vi "Demo - plot.vi"() -> ()   [LabVIEW 2021]
uses:
  Apin typedef.ctl
panel:
  in  "Analog pin":T1
  out "Waveform Chart":i32[](graph)
  out "error out":errorcluster
  in  "port":u32
  in  "Base URL":string
  in  "stop":bool
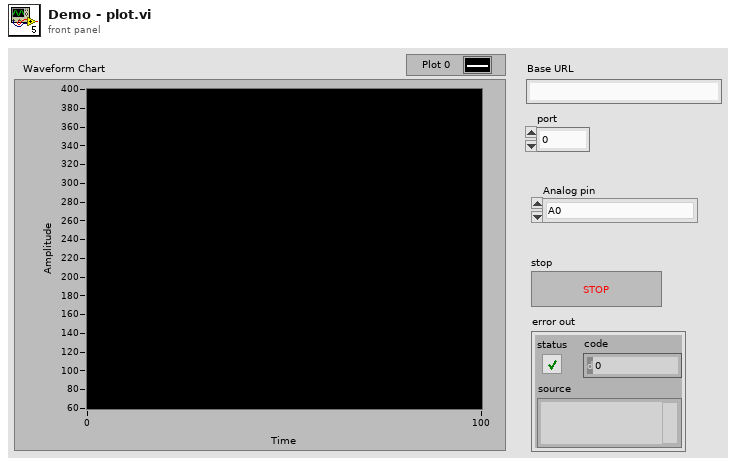
[diagram p1: front panel]
types:
  T1 = typedef "Apin typedef.ctl" = enum16{"A0", "A1", "A2", "A3", "A4", "A5"}
  T2 = typedef "UNO Q Session.ctl" = cluster{"HTTP client":T3, "Base URL":string, "Connected":bool}
  T3 = typedef "LabVIEWHTTPClient.lvlib/ClientHandle.ctl" = refnum<k1>
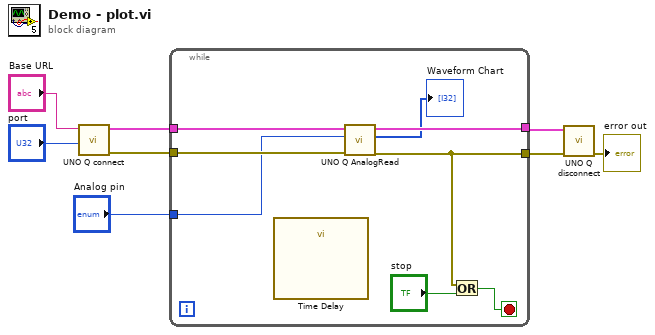
[diagram p0: block diagram]
diagram:
  n1 = call "UNO Q connect.vi"("port"="port", "Base URL"="Base URL") -> ("error out"=w5:errorcluster, "Session out"=w6:T2)  [unwired: 4 in]
  n2 = while {
    tunnel: w6 -> [w15]
    tunnel: w5 -> [w14]
    tunnel: [w16] -> w4
    tunnel: [w9] -> w2
    tunnel: "Analog pin" -> [w12]
    stop <- w11 stop-if-true
    n3 = call "Time Delay"() -> ()  [unwired: 11 in, 1 out]
    n4 = call "UNO Q AnalogRead.vi"("error in (no error)"=w14, "Analog pin"=w12, "UNO Q Session in"=w15) -> ("error out"=w9:errorcluster, "values"=→"Waveform Chart":i32[], "UNO Q Session out"=w16:T2)  [unwired: 4 in, 2 out]
    n5 = Or(x=w9, y="stop") -> (x .or. y?=w11:bool)
  }
  n6 = call "UNO Q disconnect.vi"("error in (no error)"=w2, "UNO Q Session"=w4) -> ("error out"=→"error out":errorcluster)  [unwired: 9 in]
